vi "beep_detection.vi"() -> (2 "Beep Detected!! 3":bool)   [LabVIEW 2026]
uses:
  <vilib>/sound2/lvsound2.llb/Sampling Mode.ctl
  <vilib>/sound2/lvsound2.llb/Sound Data Format.ctl
  <vilib>/sound2/lvsound2.llb/Sound Input Read (DBL).vi
  <vilib>/measure/matone.llb/Extract Single Tone Information N Chan.vi
  beepstatus.vi
  <vilib>/measure/NI_MAPro.lvlib
panel:
  out "running":bool
  in  "stop":bool
  out "Waveform Chart 2":dynamicdata(graph)
  out "detected amplitudes 5":dbl[](array[numeric]) format="%.2p"
  out "detected frequencies 5":dbl[](array[numeric]) format="%.2p"
  out "x/y 3":dbl
  in  "sound format 3":T1={"sample rate (S/s)"=22050.0, "number of channels"=2, "bits per sample"=16}
  in  "number of samples/ch 3":i32=100000
  in  "sample mode 3":T2=1 items=["Finite Samples", "Continuous Samples"]
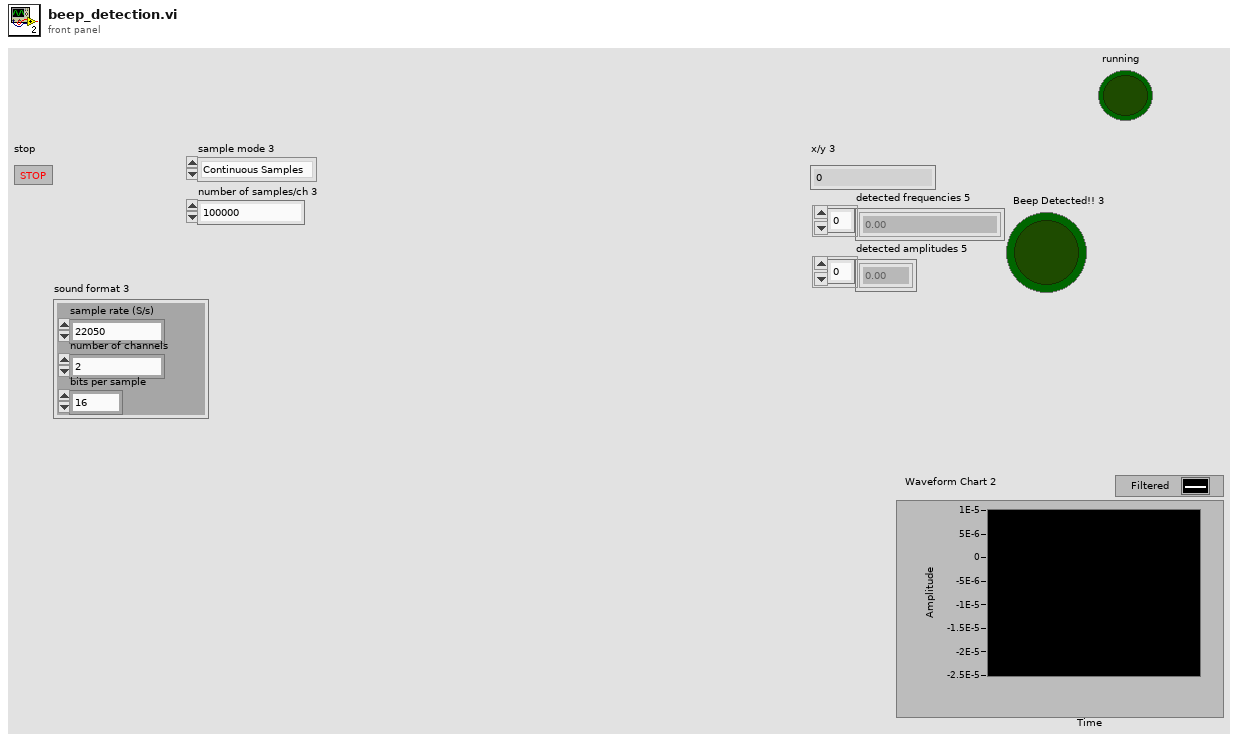
[diagram p1: front panel]
types:
  T1 = typedef "Sound Data Format.ctl" = cluster{"sample rate (S/s)":dbl, "number of channels":i32, "bits per sample":i32}
  T2 = typedef "Sampling Mode.ctl" = i32
  T3 = typedef "Sound Input Task ID.ctl" = u32
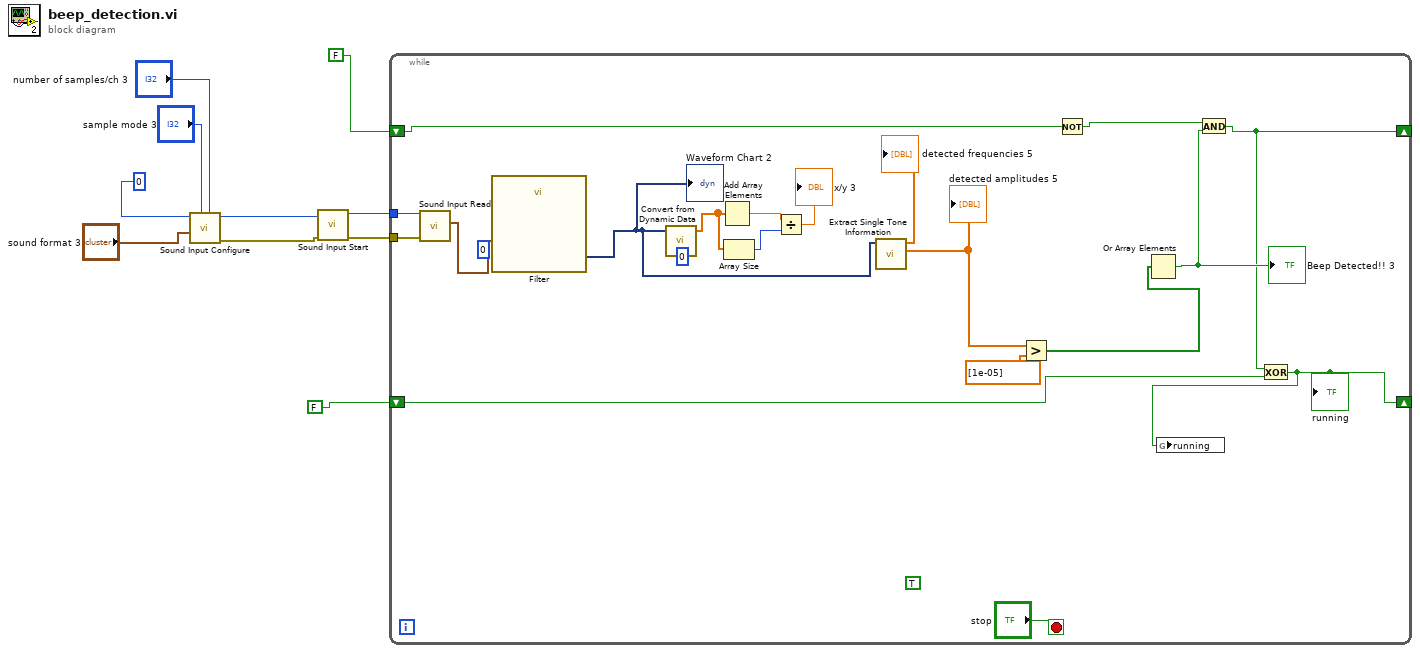
[diagram p0: block diagram]
diagram:
  n1 = call <vilib>:"Sound Input Configure.vi"("number of samples/ch"="number of samples/ch 3", "sample mode"="sample mode 3", "sound format"="sound format 3", "device ID"=u32 0) -> ("error out"=w7:errorcluster, "task ID"=w6:T3)  [unwired: 6 in]
  n2 = call <vilib>:"Sound Input Start.vi"("error in (no error)"=w7, "task ID"=w6) -> ("error out"=w4:errorcluster, "task ID out"=w3:T3)  [unwired: 8 in]
  n3 = while {
    tunnel: w4 -> [w22]
    tunnel: w3 -> [w21]
    shift-right: [w13] -> _
    shift-left: FALSE -> [w16]
    shift-right: [w11] -> _
    shift-left: FALSE -> [w12]
    stop <- "stop" stop-if-true
    (unwired) 0 ("index")
    (unwired) TRUE
    (unwired) 0 ("index")
    n4 = call-poly <vilib>:"Sound Input Read.vi"("error in (no error)"=w22, "task ID"=w21) -> ("data"=w20:waveform(dbl)[])  [unwired: 7 in, 2 out]
    n5 = call "Filter"("Signal"=w20) -> ("Filtered Signal"=w19:dynamicdata)  [unwired: 9 in, 1 out]
    "Waveform Chart 2" <- w19
    n6 = call "Convert from Dynamic Data"("Dynamic Data Type"=w19) -> ("Array"=w29:dbl[])  [unwired: 3 in]
    n7 = Add Array Elements(numeric array=w29) -> (sum=w28:dbl)
    n8 = Array Size(array=w29) -> (size(s)=w27:i32)
    n9 = Divide(x=w28, y=w27) -> (x/y=→"x/y 3":dbl)
    n10 = call-poly <vilib>:"Extract Single Tone Information.vi"("time signals in"=w19) -> ("detected amplitudes"=w24:dbl[], "detected frequencies"=→"detected frequencies 5":dbl[])  [unwired: 5 in, 4 out]
    "detected amplitudes 5" <- w24
    n11 = Greater?(x=w24, y=dbl[] [1e-05]) -> (0:w17:bool[])
    n12 = Not(x=w16) -> (.not. x?=w15:bool)
    n13 = Or Array Elements(Boolean array=w17) -> (logical OR=w14:bool)
    "Beep Detected!! 3" <- w14
    n14 = And(x=w15, y=w14) -> (x .and. y?=w13:bool)
    n15 = Exclusive Or(1:w12, 2:w13) -> (0:w11:bool)
    "running" <- w11
    n16 = global write "beepstatus.vi" "running"(w11) -> ()
  }
